vi "ALL - CalcExpress VIs.vi"() -> ()   [LabVIEW 2021]
doc: "::: CalcExpress Toolkit :::\nCopyright (c) 2000-2026 Konstantin Shifershteyn. All rights reserved."
uses:
  cetypes.llb/CalcExpress Instance RefNum.ctl
  cetypes.llb/CalcExpress Function Argument Info.ctl
panel:
  in  "False":bool
  in  "arg list":T1[](array[typedef])
  in  "CE InstanceRef":T2
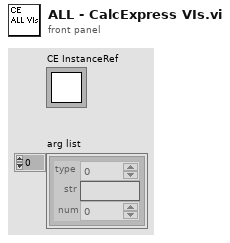
[diagram p1: front panel]
types:
  T1 = typedef "CalcExpress Function Argument Info.ctl" = cluster{"type":u32, "str":string, "num":dbl}
  T2 = typedef "CalcExpress Instance RefNum.ctl" = refnum<k1>
  T3 = cluster{"index":i32, "type":i32, "default num":dbl, "default str":string}[]
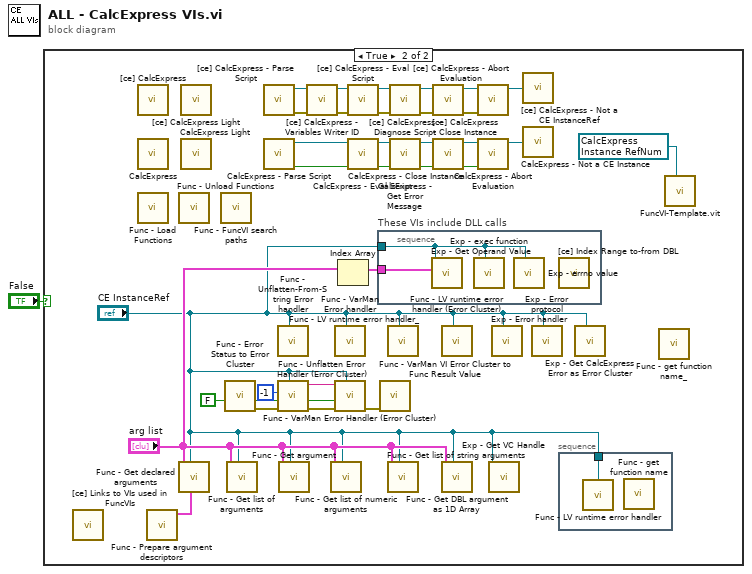
[diagram p0: block diagram]
diagram:
  n1 = case shown="True" "False" {
    frame False {
    }
    frame True {
      w16 = T2 refnum items=["CE RefNum"] ("InstanceRef")
      n2 = call "[ce] Links to VIs used in FuncVIs.vi"() -> ()  [unwired: 1 in]
      n3 = call "[ce] CalcExpress.vi"() -> ()  [unwired: 6 in, 4 out]
      n4 = call "CalcExpress.vi"() -> ()  [unwired: 7 in, 5 out]
      n5 = call "Func - Load Functions.vi"() -> ()  [unwired: 7 in, 3 out]
      n6 = call "Func - Prepare argument descriptors.vi"() -> ("arg descriptors out"=w15:T3)  [unwired: 8 in, 1 out]
      n7 = call "Func - Unload Functions.vi"() -> ()  [unwired: 9 in, 1 out]
      n8 = call "Func - Get declared arguments.vi"("arg descriptors"=w15, "InstanceRef"="CE InstanceRef", "arg list"="arg list") -> ()  [unwired: 5 in, 4 out]
      n9 = call "[ce] CalcExpress Light.vi"() -> ()  [unwired: 9 in, 3 out]
      n10 = call "CalcExpress Light.vi"() -> ()  [unwired: 8 in, 4 out]
      n11 = call "Func - FuncVI search paths.vi"() -> ()  [unwired: 6 in, 4 out]
      n12 = call "Func - Error Status to Error Cluster.vi"("error status in"=FALSE) -> ("Error Cluster out"=w4:errorcluster, "error status out"=w8:bool)  [unwired: 9 in]
      n13 = call "Func - Get list of arguments.vi"("InstanceRef"="CE InstanceRef", "arg list"="arg list") -> ()  [unwired: 6 in, 4 out]
      n14 = call "[ce] CalcExpress - Parse Script.vi"() -> ("error out"=w12:errorcluster, "CE InstanceRef"=w14:T2)  [unwired: 6 in, 2 out]
      n15 = call "CalcExpress - Parse Script.vi"() -> ("error out"=w33:bool, "CE InstanceRef"=w23:T2)  [unwired: 7 in, 3 out]
      n16 = call "Func - Unflatten-From-String Error handler.vi"("InstanceRef"="CE InstanceRef") -> ()  [unwired: 8 in, 1 out]
      n17 = call "Func - Unflatten Error Handler (Error Cluster).vi"("InstanceRef"="CE InstanceRef", "Unflatten Error Cluster"=w4, "error status before"=w8, "argument number"=-1) -> ("Error Cluster out"=w3:errorcluster, "error status out"=w9:bool, "dup name"=w10:string)  [unwired: 5 in]
      n18 = call "Func - Get argument.vi"("InstanceRef"="CE InstanceRef", "arg list"="arg list") -> ()  [unwired: 4 in, 4 out]
      n19 = call "[ce] CalcExpress - Variables Writer ID.vi"("error in"=w12, "CE InstanceRef"=w14) -> ("error out"=w11:errorcluster, "dup CE InstanceRef"=w13:T2)  [unwired: 7 in, 1 out]
      n20 = call "Func - Get list of numeric arguments.vi"("InstanceRef"="CE InstanceRef", "arg list"="arg list") -> ()  [unwired: 6 in, 2 out]
      n21 = call "Func - VarMan Error handler.vi"("InstanceRef"="CE InstanceRef") -> ()  [unwired: 6 in, 3 out]
      n22 = call "Func - VarMan Error Handler (Error Cluster).vi"("InstanceRef"="CE InstanceRef", "VarMan VI error in"=w3, "error status before"=w9, "var name"=w10) -> ("error out"=w2:errorcluster)  [unwired: 5 in, 2 out]
      n23 = Index Array(array="arg list") -> (element=w25:T1)  [unwired: 1 in]
      n24 = call "[ce] CalcExpress - Eval Script.vi"("error in"=w11, "CE InstanceRef"=w13) -> ("error out"=w19:errorcluster, "dup CE InstanceRef"=w20:T2)  [unwired: 3 in, 3 out]
      n25 = call "CalcExpress - Eval Script.vi"("error in"=w33, "CE InstanceRef"=w23) -> ("error out"=w32:bool, "dup CE InstanceRef"=w34:T2)  [unwired: 3 in, 3 out]
      n26 = stacked-sequence "These VIs include DLL calls" {
        tunnel: "CE InstanceRef" -> [w37]
        tunnel: w25 -> [w36]
        frame #0 {
          n27 = call "Exp - Get Operand Value.vi"("op info"=w36, "InstanceRef"=w37) -> ()  [unwired: 4 in, 4 out]
          n28 = call "Exp - exec function.vi"("CE InstanceRef"=w37) -> ()  [unwired: 8 in, 1 out]
          n29 = call "Exp - errno value.vi"("InstanceRef"=w37) -> ()  [unwired: 6 in, 3 out]
          n30 = call "[ce] Index Range to-from DBL.vi"() -> ()  [unwired: 10 in, 2 out]
        }
      }
      n31 = call "Func - VarMan VI Error Cluster to Func Result Value.vi"("VarMan VI error in"=w2) -> ()  [unwired: 10 in, 1 out]
      n32 = call "Func - LV runtime error handler_.vi"("InstanceRef"="CE InstanceRef") -> ()  [unwired: 10 in, 1 out]
      n33 = call "Func - Get list of string arguments.vi"("InstanceRef"="CE InstanceRef", "arg list"="arg list") -> ()  [unwired: 6 in, 2 out]
      n34 = call "[ce] CalcExpress - Diagnose Script.vi"("error in"=w19, "CE InstanceRef"=w20) -> ("error out"=w17:errorcluster, "dup CE InstanceRef"=w18:T2)  [unwired: 6 in, 2 out]
      n35 = call "CalcExpress - Get Error Message.vi"("error in"=w32, "CE InstanceRef"=w34) -> ("error out"=w31:bool, "dup CE InstanceRef"=w26:T2)  [unwired: 4 in, 2 out]
      n36 = call "[ce] CalcExpress - Close Instance.vi"("error in"=w17, "CE InstanceRef"=w18) -> ("error out"=w27:errorcluster, "dup CE InstanceRef"=w28:T2)  [unwired: 5 in, 1 out]
      n37 = call "CalcExpress - Close Instance.vi"("error in"=w31, "CE InstanceRef"=w26) -> ("error out"=w29:bool, "dup CE InstanceRef"=w30:T2)  [unwired: 5 in, 1 out]
      n38 = call "Func - LV runtime error handler (Error Cluster).vi"("InstanceRef"="CE InstanceRef") -> ()  [unwired: 5 in, 4 out]
      n39 = call "Func - Get DBL argument as 1D Array.vi"("InstanceRef"="CE InstanceRef", "arg list"="arg list") -> ()  [unwired: 6 in, 4 out]
      n40 = call "[ce] CalcExpress - Abort Evaluation.vi"("error in"=w27, "CE InstanceRef"=w28) -> ("dup CE InstanceRef"=w21:T2)  [unwired: 6 in, 1 out]
      n41 = call "CalcExpress - Abort Evaluation.vi"("error in"=w29, "CE InstanceRef"=w30) -> ("dup CE InstanceRef"=w22:T2)  [unwired: 6 in, 1 out]
      n42 = call "Exp - Get VC Handle.vi"("InstanceRef"="CE InstanceRef") -> ()  [unwired: 5 in, 4 out]
      n43 = call "Exp - Error handler.vi"("InstanceRef"="CE InstanceRef") -> ()  [unwired: 8 in, 3 out]
      n44 = call "[ce] CalcExpress - Not a CE InstanceRef.vi"("CE InstanceRef"=w21) -> ()  [unwired: 2 out]
      n45 = call "CalcExpress - Not a CE Instance.vi"("CE InstanceRef"=w22) -> ()  [unwired: 2 out]
      n46 = call "Exp - Error protocol.vi"("InstanceRef"="CE InstanceRef") -> ()  [unwired: 7 in, 2 out]
      n47 = stacked-sequence {
        tunnel: "CE InstanceRef" -> [w35]
        frame #0 {
          n48 = call "Func - LV runtime error handler.vi"("InstanceRef"=w35) -> ()  [unwired: 4 in, 1 out]
          n49 = call "Func - get function name.vi"() -> ()  [unwired: 3 in, 3 out]
        }
      }
      n50 = call "Exp - Get CalcExpress Error as Error Cluster.vi"("InstanceRef"="CE InstanceRef") -> ()  [unwired: 9 in, 2 out]
      n51 = call "Func - get function name_.vi"() -> ()  [unwired: 9 in, 3 out]
      n52 = call "FuncVI-Template.vit"("InstanceRef"=w16) -> ()  [unwired: 7 in, 2 out]
    }
  }
